vi "RP1210 Get Error Msg.vi"(8 "error in (no error)":errorcluster, 11 "ErrorCode":i16) -> (0 "error out":errorcluster, 2 "function return":i16, 3 "fpchDescription":string)   [LabVIEW 2020, in "cansub_rp1210.lvlib"]
doc: "short __stdcall RP1210_GetErrorMsg(short ErrorCode, char *fpchDescription);"
uses:
  cansub_rp1210.lvlib
  cansub_lv64.dll
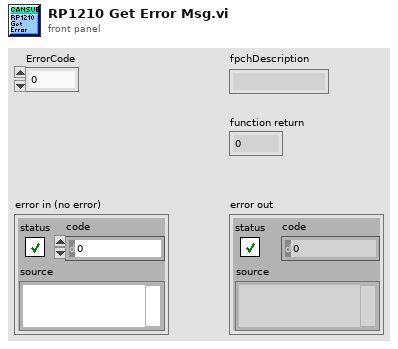
[diagram p1: front panel]
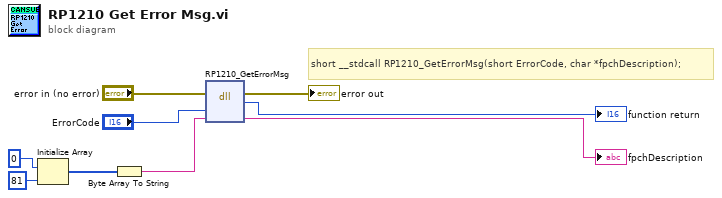
[diagram p0: block diagram]
diagram:
  # "short __stdcall RP1210_GetErrorMsg(short ErrorCode, char *fpchDescription);"
  n1 = Initialize Array(u8 0 ("element"), 81 ("dimension size")) -> (w7:u8[])
  n2 = Byte Array To String(unsigned byte array=w7) -> (string=w6:string)
  n3 = dll-call lib="C:/cansub-lv/library/cansub_lv*.*" fn="RP1210_GetErrorMsg"(error in="error in (no error)", "ErrorCode"="ErrorCode", "fpchDescription"=w6) -> (error out=→"error out":errorcluster, "return type"=→"function return":i16, "fpchDescription"=→"fpchDescription":string)  [unwired: 3 in, 1 out]
